vi "Create_Delete_User_in_program.vi"(8 "error in (no error) 3":errorcluster) -> (0 "error in (no error) 4":errorcluster)   [LabVIEW 2021]
uses:
  Control/login_type.ctl
  Control/User_login_type.ctl
  Control/add_remove.ctl
panel:
  in  "Back Button":bool
  out "Boolean 3":bool=TRUE
  out "Boolean 2":bool=TRUE
  out "Boolean":bool=TRUE
  out "Numeric":i32
  out "Enum":T1
  in  "USER TYPE":T2 items=["Admin", "Operator"]
  out "element 3":string
  out "Array 2":string[](array[string])
  in  "Remove user 3":bool
  in  "Add user  2":bool
  in  "NAME":string
  in  "PASSWORD":string
  in  "Enum":T1
  in  "error in (no error) 2":errorcluster
  in  "Multicolumn Listbox":i32(listbox)
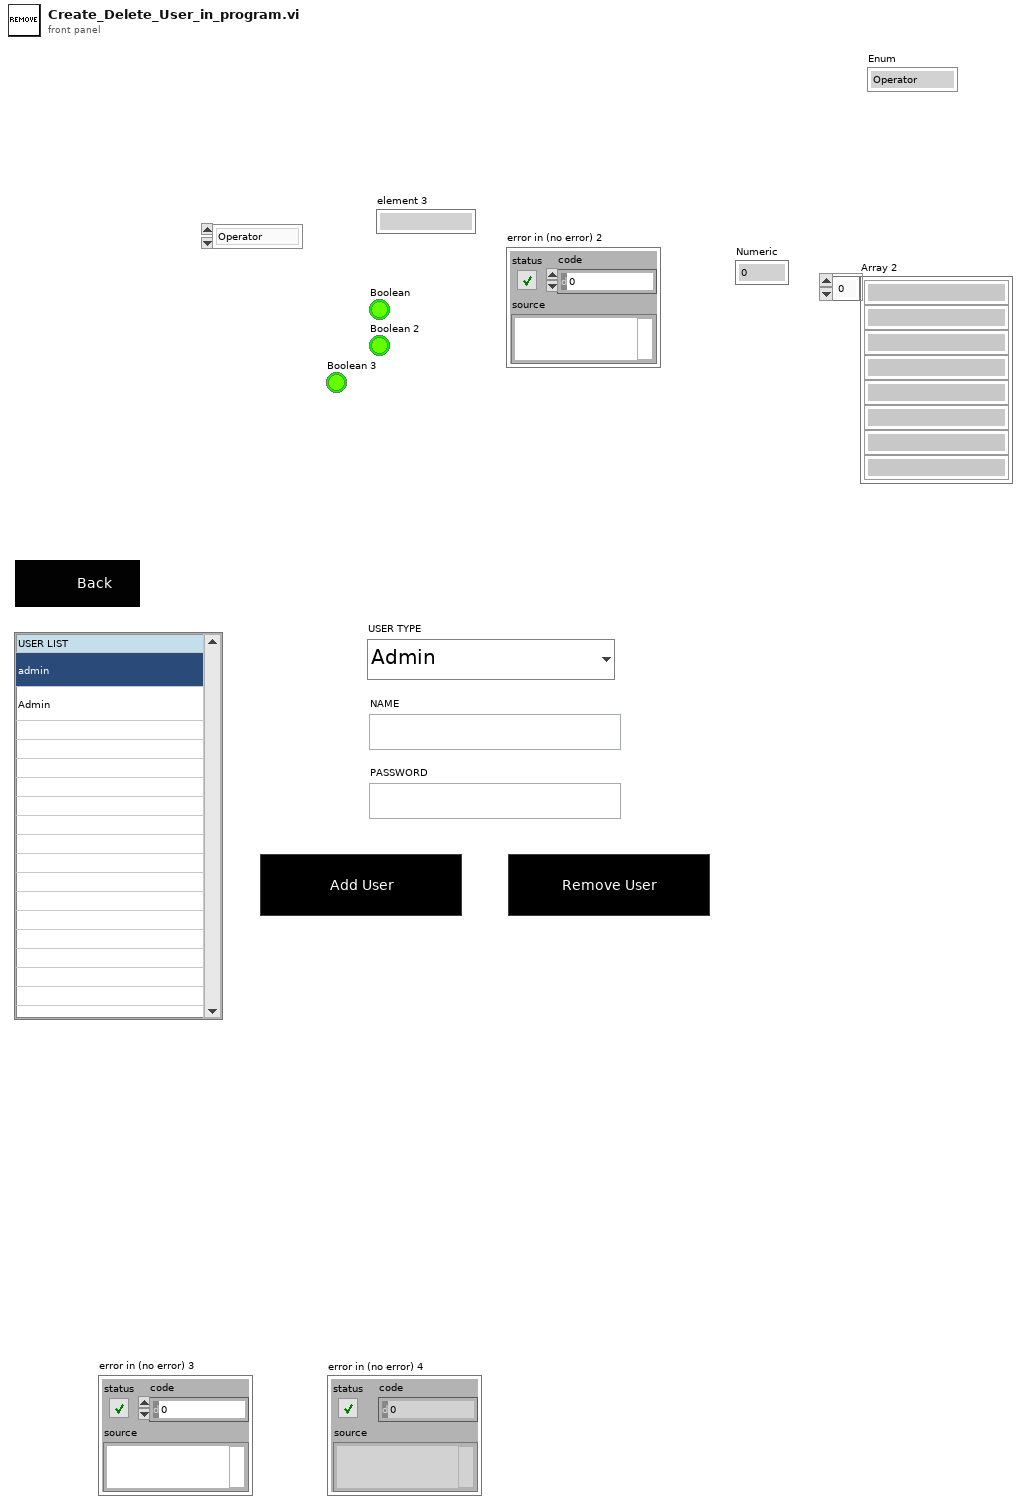
[diagram p1: front panel]
types:
  T1 = typedef "login_type.ctl" = enum16{"Operator", "Admin"}
  T2 = typedef "User_login_type.ctl" = u16
  T3 = typedef "add_remove.ctl" = enum16{"Enter", "add user", "remover user", "view user"}
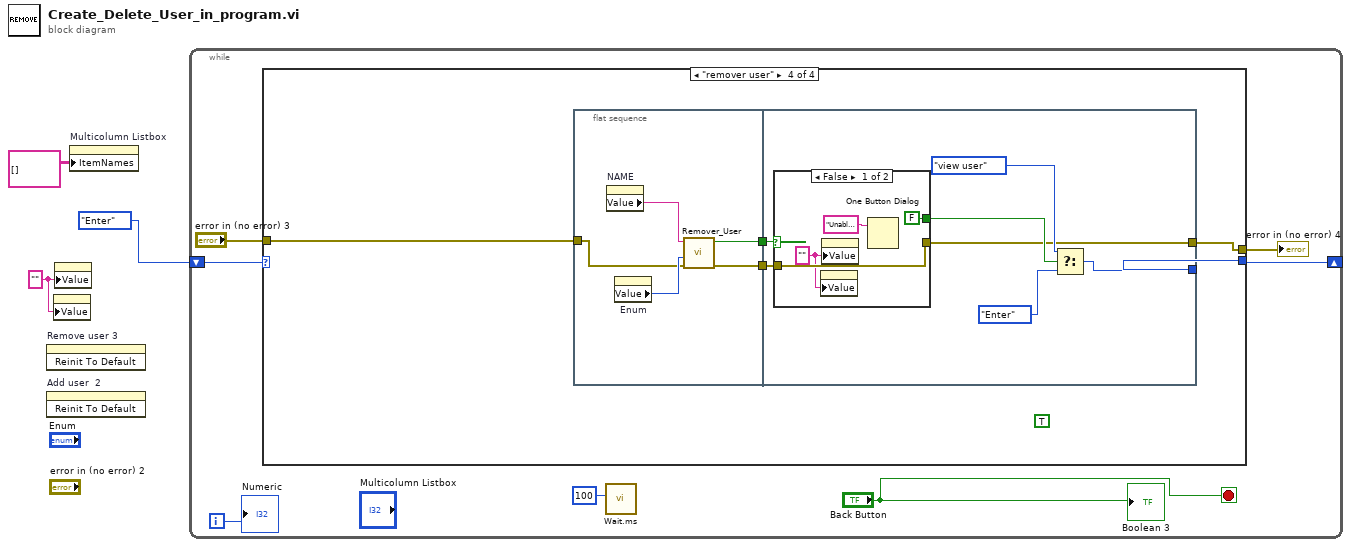
[diagram p0: block diagram]
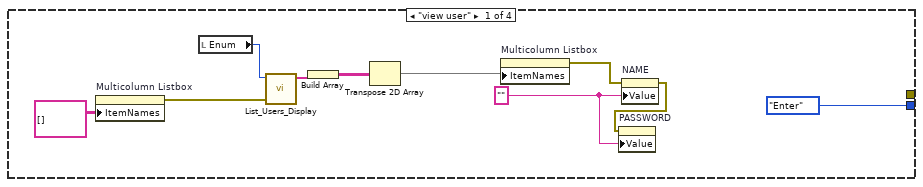
[diagram p2: hidden frame]
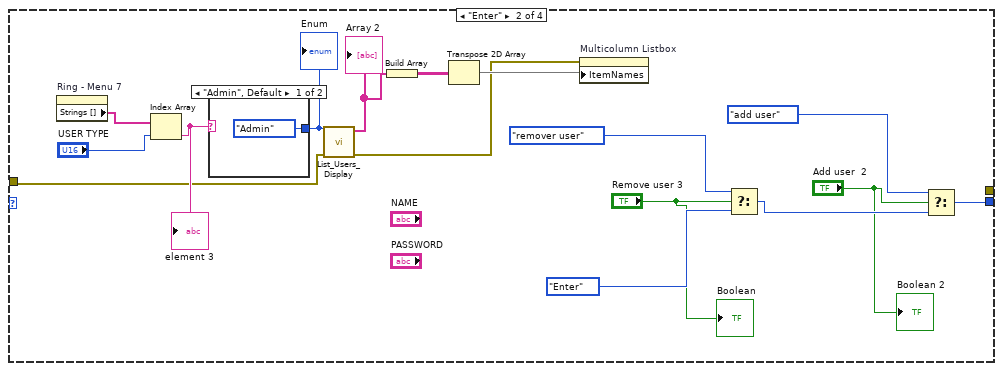
[diagram p3: hidden frame]
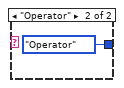
[diagram p4: hidden frame]
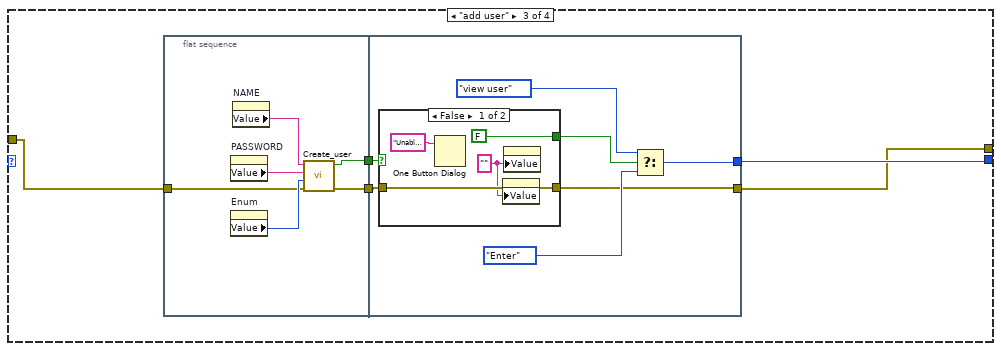
[diagram p5: hidden frame]
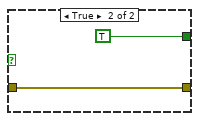
[diagram p6: hidden frame]
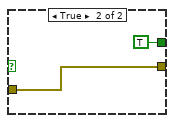
[diagram p7: hidden frame]
diagram:
  w1 = "" ("Name 3")
  n1 = invoke on="Remove user 3" class="Bool" method="Reinit To Default"() -> ()  [unwired: 3 in, 3 out]
  n2 = invoke on="Add user  2" class="Bool" method="Reinit To Default"() -> ()  [unwired: 3 in, 3 out]
  n3 = property on="PASSWORD" class="Str"("Value"=w1) -> ()  [unwired: 2 in, 2 out]
  n4 = property on="NAME" class="Str"("Value"=w1) -> ()  [unwired: 2 in, 2 out]
  n5 = property on="Multicolumn Listbox" class="MCListbox (strict)"("ItemNames"=string[][] [] ("Item Names")) -> ()  [unwired: 2 in, 2 out]
  n6 = while {
    shift-right: [w9] -> _
    shift-left: add_remove."Enter" -> [w10]
    i -> [w8]
    stop <- "Back Button" stop-if-true
    n7 = case shown="\"remover user\"" w10 {
      tunnel: [add_remove."Enter" ("f") w32 w41 w64] -> w9
      tunnel: "error in (no error) 3" -> [_ w22 w43 w67]
      tunnel: [_ _ w39 w63] -> w5
      frame "view user" {
        w13 = "" ("Name 3")
        n8 = property on="Multicolumn Listbox" class="MCListbox (strict)"("ItemNames"=string[][] [] ("Item Names")) -> (error out=w15:errorcluster)  [unwired: 2 in, 1 out]
        n9 = local read "Enum"() -> (w20:T1)
        n10 = call "List_Users_Display.vi"("error in (no error)"=w15, "Enum"=w20) -> ("Array"=w17:string[])  [unwired: 8 in, 1 out]
        n11 = Build Array(w17) -> (w19:string[][])
        n12 = Transpose 2D Array(2D array=w19) -> (transposed array=w18:string[][])
        n13 = property on="Multicolumn Listbox" class="MCListbox (strict)"("ItemNames"=w18) -> (error out=w12:errorcluster)  [unwired: 2 in, 1 out]
        n14 = property on="NAME" class="Str"(error in=w12, "Value"=w13) -> (error out=w11:errorcluster)  [unwired: 1 in, 1 out]
        n15 = property on="PASSWORD" class="Str"(error in=w11, "Value"=w13) -> ()  [unwired: 1 in, 2 out]
      }
      frame "Enter" {
        n16 = property on="Ring - Menu 7" class="Ring (strict)"() -> ("Strings []"=w36:string[])  [unwired: 2 in, 2 out]
        n17 = Index Array(array=w36, index="USER TYPE") -> (element=w34:string)
        "element 3" <- w34
        n18 = case shown="\"Admin\", Default" w34 {
          tunnel: [login_type."Admin" login_type."Operator"] -> w33
          frame "Admin", Default {
          }
          frame "Operator" {
          }
        }
        "Enum" <- w33
        n19 = call "List_Users_Display.vi"("error in (no error)"=w22, "Enum"=w33) -> ("error out"=w21:errorcluster, "Array"=w30:string[])  [unwired: 8 in]
        "Array 2" <- w30
        n20 = Build Array(w30) -> (w29:string[][])
        n21 = Transpose 2D Array(2D array=w29) -> (transposed array=w28:string[][])
        n22 = property on="Multicolumn Listbox" class="MCListbox (strict)"(error in=w21, "ItemNames"=w28) -> ()  [unwired: 1 in, 2 out]
        n23 = Select(t=add_remove."remover user", s="Remove user 3", f=add_remove."Enter") -> (s? t:f=w31:T3)
        n24 = Select(t=add_remove."add user", s="Add user  2", f=w31) -> (s? t:f=w32:T3)
        "Boolean" <- "Remove user 3"
        "Boolean 2" <- "Add user  2"
      }
      frame "add user" {
        n25 = flat-sequence {
          tunnel: w43 -> [w45]
          tunnel: [w49] -> w42
          tunnel: [w44] -> w40
          tunnel: w42 -> [w53]
          tunnel: [w54] -> w41
          tunnel: w40 -> [w51]
          tunnel: [w50] -> w39
          frame #0 {
            n26 = property on="PASSWORD" class="Str"() -> ("Value"=w47:string)  [unwired: 2 in, 2 out]
            n27 = property on="Enum" class="Enum (strict)"() -> ("Value"=w46:T1)  [unwired: 2 in, 2 out]
            n28 = property on="NAME" class="Str"() -> ("Value"=w48:string)  [unwired: 2 in, 2 out]
            n29 = call "Create_user.vi"("error in (no error)"=w45, "Enum"=w46, "Password"=w47, "Name"=w48) -> ("error out"=w44:errorcluster, "Result"=w49:bool)  [unwired: 6 in]
          }
          frame #1 {
            n30 = case shown="False" w53 {
              tunnel: [FALSE TRUE] -> w52
              tunnel: w51 -> [w58 w62]
              tunnel: [w58 w62] -> w50
              frame False {
                w57 = "" ("Name 3")
                n31 = One Button Dialog(message="Unable to add the user") -> ()  [unwired: 1 in, 1 out]
                n32 = property on="PASSWORD" class="Str"("Value"=w57) -> ()  [unwired: 2 in, 2 out]
                n33 = property on="NAME" class="Str"("Value"=w57) -> ()  [unwired: 2 in, 2 out]
              }
              frame True {
              }
            }
            n34 = Select(t=add_remove."view user", s=w52, f=add_remove."Enter") -> (s? t:f=w54:T3)
          }
        }
      }
      frame "remover user" {
        (unwired) TRUE
        n35 = flat-sequence {
          tunnel: w67 -> [w69]
          tunnel: [w72] -> w66
          tunnel: [w68] -> w65
          tunnel: w66 -> [w76]
          tunnel: w65 -> [w74]
          tunnel: [w77] -> w64
          tunnel: [w73] -> w63
          frame #0 {
            n36 = property on="NAME" class="Str"() -> ("Value"=w71:string)  [unwired: 2 in, 2 out]
            n37 = property on="Enum" class="Enum (strict)"() -> ("Value"=w70:T1)  [unwired: 2 in, 2 out]
            n38 = call "Remover_User.vi"("error in (no error)"=w69, "Enum"=w70, "Name"=w71) -> ("error out"=w68:errorcluster, "Result"=w72:bool)  [unwired: 7 in]
          }
          frame #1 {
            n39 = case shown="False" w76 {
              tunnel: [FALSE TRUE] -> w75
              tunnel: w74 -> [w81 w85]
              tunnel: [w81 w85] -> w73
              frame False {
                w80 = "" ("Name 3")
                n40 = property on="PASSWORD" class="Str"("Value"=w80) -> ()  [unwired: 2 in, 2 out]
                n41 = property on="NAME" class="Str"("Value"=w80) -> ()  [unwired: 2 in, 2 out]
                n42 = One Button Dialog(message="Unable to Remove the user") -> ()  [unwired: 1 in, 1 out]
              }
              frame True {
              }
            }
            n43 = Select(t=add_remove."view user", s=w75, f=add_remove."Enter") -> (s? t:f=w77:T3)
          }
        }
      }
    }
    "error in (no error) 4" <- w5
    n44 = call "Wait.ms.vi"("milliseconds to wait"=u32 100) -> ()  [unwired: 10 in, 1 out]
    "Numeric" <- w8
    "Boolean 3" <- "Back Button"
  }
